vi "关闭引用.vi"(8 "错误输入（无错误）":errorcluster, 10 "引用":refnum<vi>) -> (0 "错误输出":errorcluster)   [LabVIEW 2026, in "UI-Zolix.lvlib"]
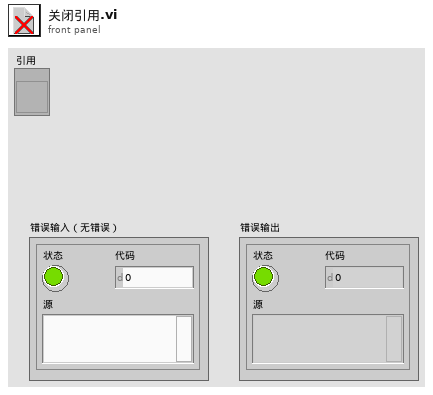
[diagram p1: front panel]
types:
  T1 = enum32{"Bad", "Idle", "Run top level", "Running"}
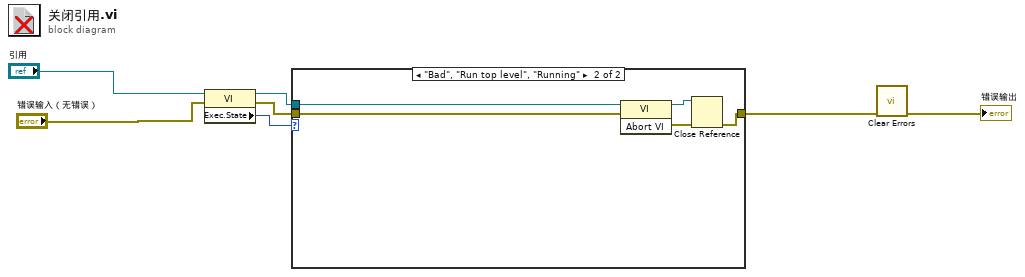
[diagram p0: block diagram]
diagram:
  n1 = property class="VI"(reference="引用", error in="错误输入（无错误）") -> (reference out=w4:refnum<vi>, error out=w6:errorcluster, "Exec.State"=w5:T1)
  n2 = case shown="\"Bad\", \"Run top level\", \"Running\"" w5 {
    tunnel: w6 -> [w8 w10]
    tunnel: [w8 w13] -> w7
    tunnel: w4 -> [_ w9]
    frame "Idle" {
    }
    frame "Bad", "Run top level", "Running" {
      n3 = invoke on="Invoke Node" class="VI" method="Abort VI"(reference=w9, error in=w10) -> (reference out=w11:refnum<vi>, error out=w12:errorcluster)  [unwired: 1 in, 1 out]
      n4 = Close Reference(reference=w11, error in (no error)=w12) -> (error out=w13:errorcluster)
    }
  }
  n5 = call <vilib>:"Clear Errors.vi"("error in (no error)"=w7) -> ("error out"=→"错误输出":errorcluster)  [unwired: 5 in, 1 out]
